vi "SetTestv1NoRbac.vi"() -> ()   [LabVIEW 2017]
uses:
  <userlib>/_RADE/japc/classes/JSet/JSet.lvclass
  <vilib>/Analysis/NI_AALBase.lvlib
panel:
  out "standard deviation":dbl format="%0.2f"
  out "mean":dbl format="%0.2f"
  out "error out":errorcluster
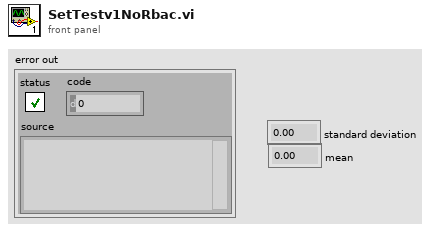
[diagram p1: front panel]
types:
  T1 = cluster{"dbl_field":dbl, "string_field":string, "long_field":i64, "int_array_field":i32[]}
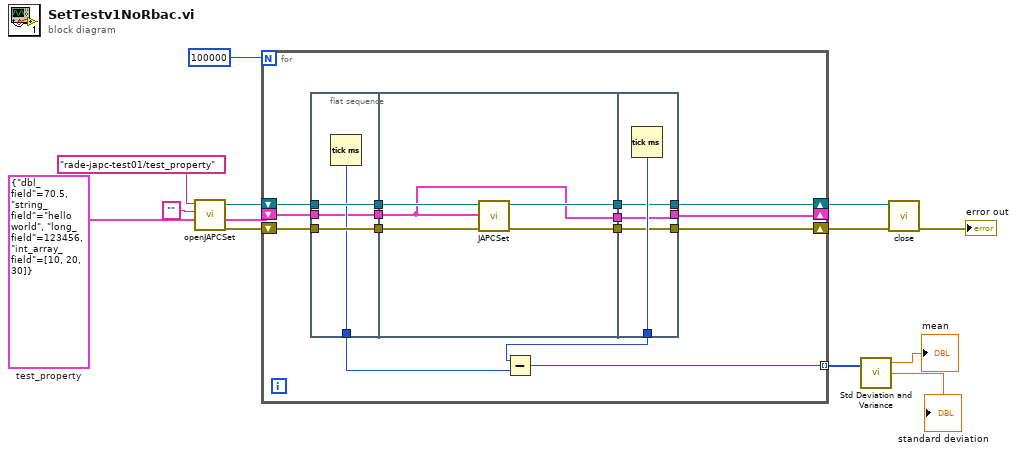
[diagram p0: block diagram]
diagram:
  w4 = T1 {"dbl_field"=70.5, "string_field"="hello world", "long_field"=123456, "int_array_field"=[10, 20, 30]}  # test_property
  n1 = call <userlib>:"openJAPCSet.vi"("Data type"=w4, "Cycle"="", "URL"="rade-japc-test01/test_property") -> ("error out"=w5:errorcluster, "Object out"=w6:refnum<class "JSet.lvclass">)  [unwired: 7 in]
  n2 = for {
    N: 100000 -> [_]
    tunnel: [w23] -> w10 mode=indexing
    shift-right: [w17] -> w8
    shift-left: w5 -> [w24]
    shift-right: [w19] -> w7
    shift-left: w6 -> [w26]
    shift-right: [w14] -> _
    shift-left: w4 -> [w15]
    n3 = flat-sequence {
      tunnel: [w31] -> w27
      tunnel: w26 -> [w31]
      tunnel: [w30] -> w25
      tunnel: w24 -> [w30]
      tunnel: [w29] -> w22
      tunnel: [w28] -> w16
      tunnel: w15 -> [w28]
      tunnel: w27 -> [w33]
      tunnel: w25 -> [w34]
      tunnel: [w36] -> w20
      tunnel: [w35] -> w18
      tunnel: w16 -> [w32]
      tunnel: [w32] -> w13
      tunnel: [w40] -> w21
      tunnel: [w39] -> w19
      tunnel: w20 -> [w39]
      tunnel: [w38] -> w17
      tunnel: w18 -> [w38]
      tunnel: [w37] -> w14
      tunnel: w13 -> [w37]
      frame #0 {
        n4 = Tick Count (ms)() -> (millisecond timer value=w29:u32)
      }
      frame #1 {
        n5 = call <userlib>:"JAPCSet.vi"("error in (no error)"=w34, "Data"=w32, "Object in"=w33) -> ("error out"=w35:errorcluster, "Object out"=w36:refnum<class "JSet.lvclass">)  [unwired: 7 in]
      }
      frame #2 {
        n6 = Tick Count (ms)() -> (millisecond timer value=w40:u32)
      }
    }
    n7 = Subtract(x=w21, y=w22) -> (x-y=w23:u32)
  }
  n8 = call <vilib>:"Std Deviation and Variance.vi"("X"=w10) -> ("mean"=→"mean":dbl, "standard deviation"=→"standard deviation":dbl)  [unwired: 1 in, 1 out]
  n9 = call-dynamic "close.vi"("error in (no error)"=w8, "Object in"=w7) -> ("error out"=→"error out":errorcluster)  [unwired: 9 in]
